vi "FSK Main.vi"() -> ()   [LabVIEW 2026]
panel:
  out "FSK Modulated Signal":dbl[](graph)
  out "Baseband Signal":dbl[](graph)
  out "Recovered Binary Signal":dbl[](array[numeric])
  in  "Lower Frequency (f0)":dbl
  in  "Higher Frequency(f1)":dbl
  in  "Carrier Amplitude(A)":dbl
  in  "Bit Rate(Rb)":dbl
  in  "Binary Input":i32[](array[numeric])
  in  "Sampling Frequency(Fs)":dbl
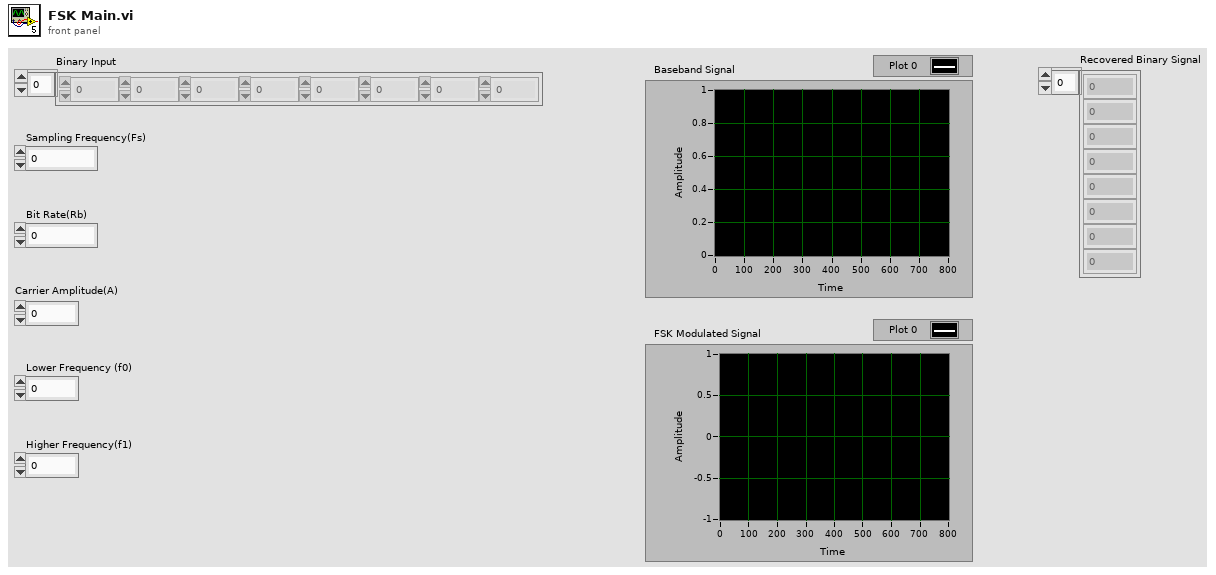
[diagram p1: front panel]
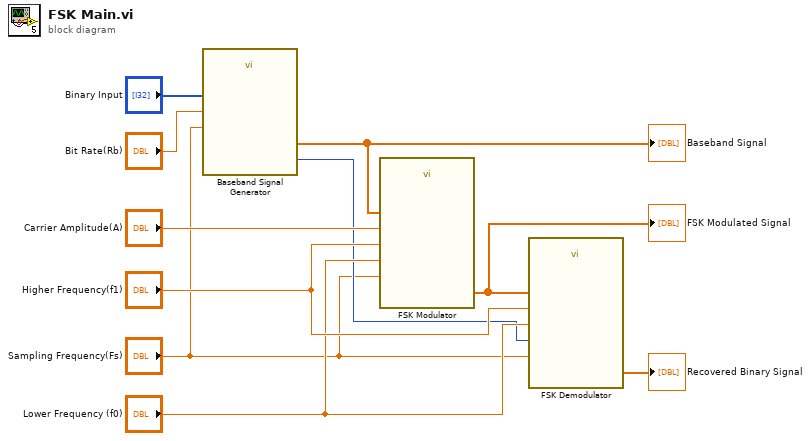
[diagram p0: block diagram]
diagram:
  n1 = call "Baseband Signal Generator.vi"("Bit Rate(Rb)"="Bit Rate(Rb)", "Sampling Frequency(Fs)"="Sampling Frequency(Fs)", "Binary Input"="Binary Input") -> ("Baseband Signal"=w2:dbl[], "Samples per bit"=w5:i32)
  "Baseband Signal" <- w2
  n2 = call "FSK Modulator.vi"("Baseband Signal"=w2, "Sampling Frequency(Fs)"="Sampling Frequency(Fs)", "Lower Frequency (f0)"="Lower Frequency (f0)", "Higher Frequency(f1)"="Higher Frequency(f1)", "Carrier Amplitude(A)"="Carrier Amplitude(A)") -> ("FSK Modulated Signal"=w1:dbl[])
  "FSK Modulated Signal" <- w1
  n3 = call "FSK Demodulator.vi"("FSK Modulated Signal"=w1, "Sampling Frequency (Fs)"="Sampling Frequency(Fs)", "Lower Frequency (f0)"="Lower Frequency (f0)", "Higher Frequency (f1)"="Higher Frequency(f1)", "Samples per Bit"=w5) -> ("Recovered Binary Signal"=→"Recovered Binary Signal":dbl[])
